vi "十字路口仿真V3.0.vi"() -> ()   [LabVIEW 2014]
panel:
  out "PW_N_R":bool
  out "PW_S_R":bool
  out "PW_E_R":bool
  out "PW_W_R":bool
  out "PW_N_G":bool
  out "PW_S_G":bool
  out "PW_E_G":bool
  out "PW_W_G":bool
  out "BK_NS_TH_R":bool
  out "BK_NS_LT_R":bool
  out "BK_EW_TH_R":bool
  out "BK_EW_LT_R":bool
  out "BK_NS_TH_G":bool
  out "BK_NS_LT_G":bool
  out "BK_EW_TH_G":bool
  out "BK_EW_LT_G":bool
  out "loop_count":dbl
  in  "停止":bool
  in  "step_ms":dbl
  out "slice_name":string
  out "cycle_no":dbl
  out "remain_s":dbl
  out "t_s":dbl
  out "EW_LT_G":bool
  out "EW_TH_G":bool
  out "NS_LT_G":bool
  out "NS_TH_G":bool
  out "EW_LT_Y":bool
  out "EW_TH_Y":bool
  out "NS_LT_Y":bool
  out "NS_TH_Y":bool
  out "EW_LT_R":bool
  out "EW_TH_R":bool
  out "NS_LT_R":bool
  out "NS_TH_R":bool
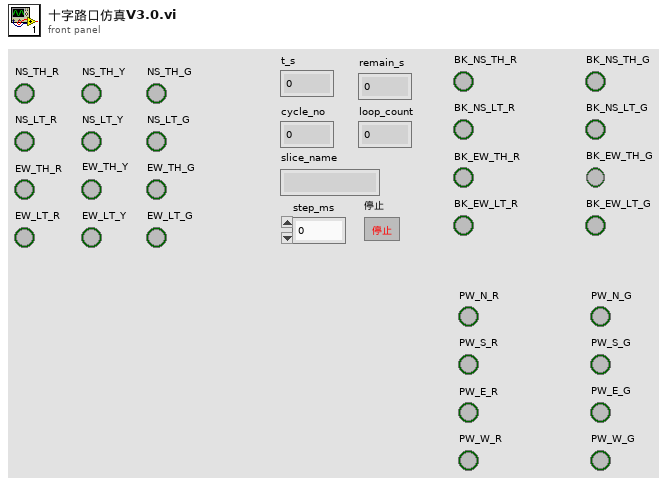
[diagram p1: front panel]
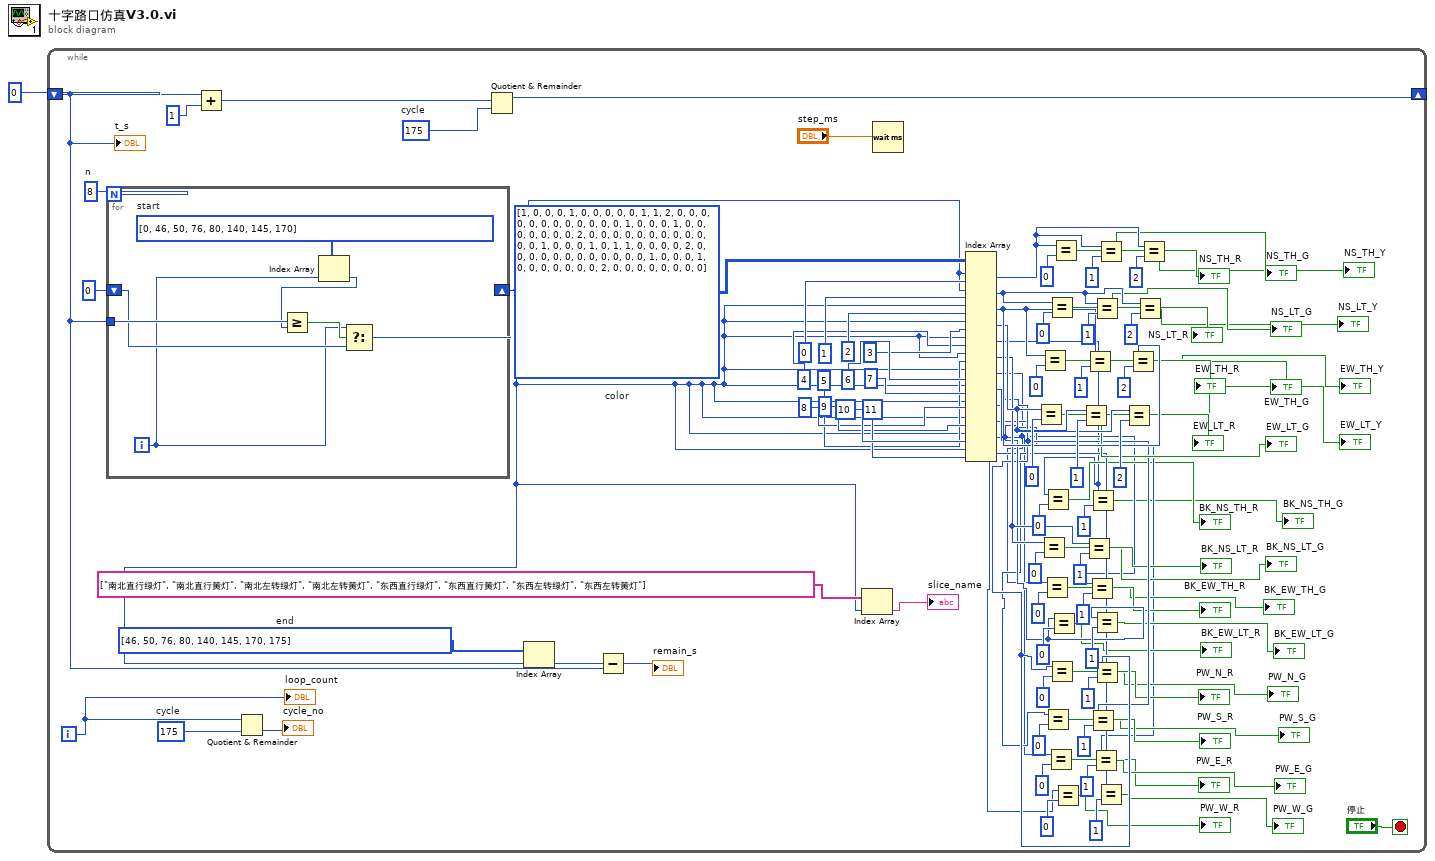
[diagram p0: block diagram]
diagram:
  n1 = while {
    shift-right: [w96] -> _
    shift-left: 0 -> [w58]
    i -> [w53]
    stop <- "停止" stop-if-true
    w55 = 175  # cycle
    w61 = i32[] [46, 50, 76, 80, 140, 145, 170, 175]  # end
    w81 = i32[][] [[1, 0, 0, 0, 1, 0, 0, 0, 0, 0, 1, 1], [2, 0, 0, 0, 0, 0, 0, 0, 0, 0, 0, 0], [0, 1, 0, 0, 0, 1, 0, 0, 0, 0, 0, 0], [0, 2, 0, 0, 0, 0, 0, 0, 0, 0, 0, 0], [0, 0, 1, 0, 0, 0, 1, 0, 1, 1, 0, 0], [0, 0, 2, 0, 0, 0, 0, 0, 0, 0, 0, 0], [0, 0, 0, 1, 0, 0, 0, 1, 0, 0, 0, 0], [0, 0, 0, 2, 0, 0, 0, 0, 0, 0, 0, 0]]  # color
    w95 = 8  # n
    w97 = 175  # cycle
    n2 = for {
      N: w95 -> [_]
      shift-right: [w103] -> w3
      shift-left: 0 -> [w104]
      tunnel: w58 -> [w106]
      i -> [w101]
      w107 = i32[] [0, 46, 50, 76, 80, 140, 145, 170]  # start
      n3 = Index Array(array=w107, index=w101) -> (element=w102:i32)
      n4 = Greater Or Equal?(x=w106, y=w102) -> (x >= y?=w105:bool)
      n5 = Select(t=w101, s=w105, f=w104) -> (s? t:f=w103:i32)
    }
    n6 = Add(x=w58, y=1) -> (x+y=w98:i32)
    n7 = Quotient & Remainder(x=w53, y=w55) -> (floor(x/y)=→"cycle_no":i32)  [unwired: 1 out]
    n8 = Quotient & Remainder(x=w98, y=w97) -> (x-y*floor(x/y)=w96:i32)  [unwired: 1 out]
    n9 = Index Array(array=w61, index=w3) -> (element=w60:i32)
    n10 = Subtract(x=w60, y=w58) -> (x-y=→"remain_s":i32)
    n11 = Index Array(array=string[] ["南北直行绿灯", "南北直行黄灯", "南北左转绿灯", "南北左转黄灯", "东西直行绿灯", "东西直行黄灯", "东西左转绿灯", "东西左转黄灯"], index=w3) -> (element=→"slice_name":string)
    n12 = Wait (ms)(milliseconds to wait="step_ms") -> ()  [unwired: 1 out]
    n13 = Index Array(array=w81, index (row) #1=w3, index (col) #1=0, index (row) #2=w3, index (col) #2=1, index (row) #3=w3, index (col) #3=2, index (row) #4=w3, index (col) #4=3, index (row) #5=w3, index (col) #5=4, index (row) #6=w3, index (col) #6=5, index (row) #7=w3, index (col) #7=6, index (row) #8=w3, index (col) #8=7, index (row) #9=w3, index (col) #9=8, index (row) #10=w3, index (col) #10=9, index (row) #11=w3, index (col) #11=10, index (row) #12=w3, index (col) #12=11) -> (element #1=w77:i32, element #2=w76:i32, element #3=w75:i32, element #4=w74:i32, element #5=w2:i32, element #6=w31:i32, element #7=w8:i32, element #8=w30:i32, element #9=w29:i32, element #10=w28:i32, element #11=w11:i32, element #12=w27:i32)
    n14 = Equal?(x=w74, y=0) -> (x = y?=→"EW_LT_R":bool)
    n15 = Equal?(x=w31, y=0) -> (x = y?=→"BK_NS_LT_R":bool)
    n16 = Equal?(x=w75, y=0) -> (x = y?=→"EW_TH_R":bool)
    n17 = Equal?(x=w8, y=0) -> (x = y?=→"BK_EW_TH_R":bool)
    n18 = Equal?(x=w2, y=0) -> (x = y?=→"BK_NS_TH_R":bool)
    n19 = Equal?(x=w28, y=0) -> (x = y?=→"PW_S_R":bool)
    n20 = Equal?(x=w11, y=0) -> (x = y?=→"PW_E_R":bool)
    n21 = Equal?(x=w76, y=0) -> (x = y?=→"NS_LT_R":bool)
    n22 = Equal?(x=w29, y=0) -> (x = y?=→"PW_N_R":bool)
    n23 = Equal?(x=w30, y=0) -> (x = y?=→"BK_EW_LT_R":bool)
    n24 = Equal?(x=w77, y=0) -> (x = y?=→"NS_TH_R":bool)
    n25 = Equal?(x=w27, y=0) -> (x = y?=→"PW_W_R":bool)
    n26 = Equal?(x=w74, y=1) -> (x = y?=→"EW_LT_G":bool)
    n27 = Equal?(x=w31, y=1) -> (x = y?=→"BK_NS_LT_G":bool)
    n28 = Equal?(x=w75, y=1) -> (x = y?=→"EW_TH_G":bool)
    n29 = Equal?(x=w8, y=1) -> (x = y?=→"BK_EW_TH_G":bool)
    n30 = Equal?(x=w2, y=1) -> (x = y?=→"BK_NS_TH_G":bool)
    n31 = Equal?(x=w28, y=1) -> (x = y?=→"PW_S_G":bool)
    n32 = Equal?(x=w11, y=1) -> (x = y?=→"PW_E_G":bool)
    n33 = Equal?(x=w76, y=1) -> (x = y?=→"NS_LT_G":bool)
    n34 = Equal?(x=w30, y=1) -> (x = y?=→"BK_EW_LT_G":bool)
    n35 = Equal?(x=w29, y=1) -> (x = y?=→"PW_N_G":bool)
    n36 = Equal?(x=w77, y=1) -> (x = y?=→"NS_TH_G":bool)
    n37 = Equal?(x=w27, y=1) -> (x = y?=→"PW_W_G":bool)
    n38 = Equal?(x=w74, y=2) -> (x = y?=→"EW_LT_Y":bool)
    n39 = Equal?(x=w75, y=2) -> (x = y?=→"EW_TH_Y":bool)
    n40 = Equal?(x=w76, y=2) -> (x = y?=→"NS_LT_Y":bool)
    n41 = Equal?(x=w77, y=2) -> (x = y?=→"NS_TH_Y":bool)
    "t_s" <- w58
    "loop_count" <- w53
  }
